vi "Get Page VI.vi"(8 "error in (no error)":errorcluster, 9 "GUID":string, 10 "Item Ref":T1 format="%.0x", 11 "System Explorer Dispatcher Implementation in":refnum<class "System Explorer Dispatcher.lvclass">) -> (0 "error out":errorcluster, 2 "page reference":refnum<vi>, 3 "System Explorer Dispatcher Implementation out":refnum<class "System Explorer Dispatcher.lvclass">)   [LabVIEW 2020, in "AIM ARINC 429 System Explorer.lvlib" / "Implementation.lvlib" / "System Explorer Dispatcher.lvclass"]
uses:
  System Explorer Dispatcher.lvclass
  <vilib>/NI VeriStand/Custom Device API/Custom Device Item Ref.ctl
  Scripting/AIM/Constants.vi
  System Explorer/Pages/Timing.vi
  Implementation.lvlib
  Scripting/AIM/AIM ARINC 429 Scripting.lvlib
  <vilib>/NI VeriStand/Custom Device API/Custom Device API.lvlib
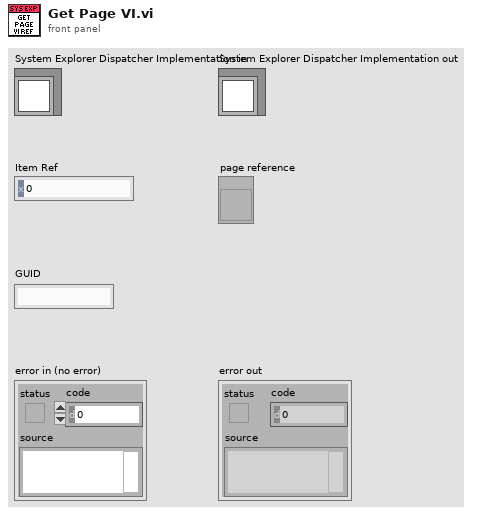
[diagram p1: front panel]
types:
  T1 = typedef "Custom Device API.lvlib/Custom Device Item Ref.ctl" = u64
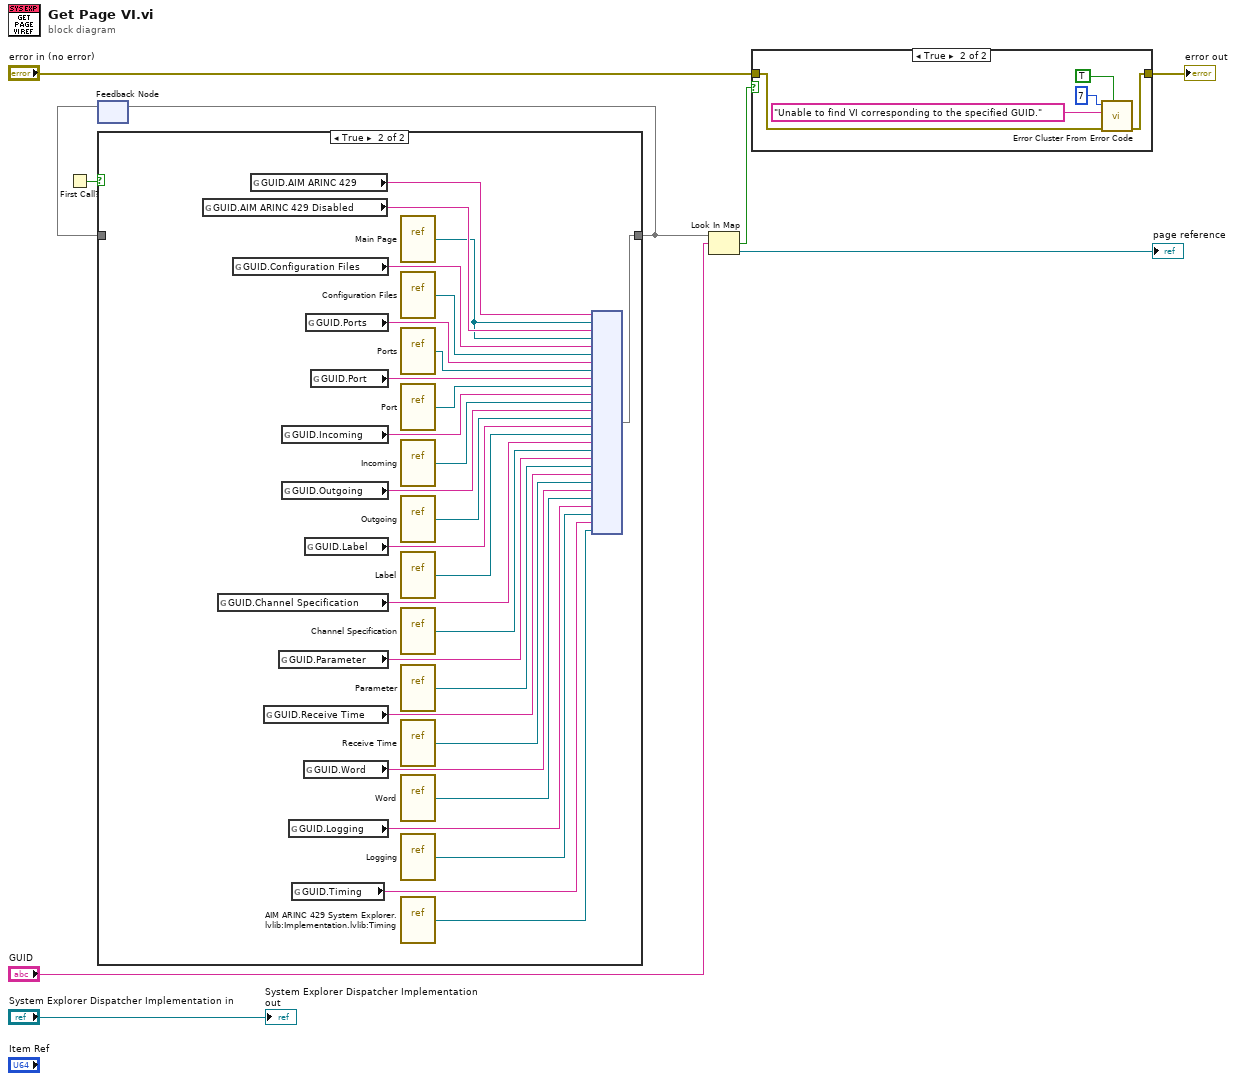
[diagram p0: block diagram]
diagram:
  n1 = First Call?() -> (First Call?: T/F=w8:bool)
  n2 = feedback #1() -> (w7:map{string, refnum<vi>})  [unwired: 1 in]
  n3 = case shown="True" w8 {
    tunnel: [w10 w38] -> w6
    tunnel: w7 -> [w10 _]
    frame False {
    }
    frame True {
      n4 = global read "Constants.vi" "GUID.AIM ARINC 429 Disabled"() -> (w16:string)
      n5 = global read "Constants.vi" "GUID.Channel Specification"() -> (w25:string)
      n6 = global read "Constants.vi" "GUID.Configuration Files"() -> (w36:string)
      n7 = global read "Constants.vi" "GUID.AIM ARINC 429"() -> (w17:string)
      n8 = global read "Constants.vi" "GUID.Receive Time"() -> (w21:string)
      n9 = global read "Constants.vi" "GUID.Parameter"() -> (w23:string)
      n10 = global read "Constants.vi" "GUID.Incoming"() -> (w31:string)
      n11 = global read "Constants.vi" "GUID.Outgoing"() -> (w29:string)
      n12 = global read "Constants.vi" "GUID.Logging"() -> (w14:string)
      n13 = global read "Constants.vi" "GUID.Timing"() -> (w12:string)
      n14 = global read "Constants.vi" "GUID.Word"() -> (w19:string)
      n15 = global read "Constants.vi" "GUID.Label"() -> (w27:string)
      n16 = global read "Constants.vi" "GUID.Ports"() -> (w35:string)
      n17 = global read "Constants.vi" "GUID.Port"() -> (w33:string)
      n18 = vi-ref "Main Page.vi"() -> (w15:refnum<vi>)
      n19 = vi-ref "Configuration Files.vi"() -> (w37:refnum<vi>)
      n20 = vi-ref "Ports.vi"() -> (w34:refnum<vi>)
      n21 = vi-ref "Port.vi"() -> (w32:refnum<vi>)
      n22 = vi-ref "Incoming.vi"() -> (w30:refnum<vi>)
      n23 = vi-ref "Outgoing.vi"() -> (w28:refnum<vi>)
      n24 = vi-ref "Label.vi"() -> (w26:refnum<vi>)
      n25 = vi-ref "Channel Specification.vi"() -> (w24:refnum<vi>)
      n26 = vi-ref "Parameter.vi"() -> (w22:refnum<vi>)
      n27 = vi-ref "Receive Time.vi"() -> (w20:refnum<vi>)
      n28 = vi-ref "Word.vi"() -> (w18:refnum<vi>)
      n29 = vi-ref "Logging.vi"() -> (w13:refnum<vi>)
      n30 = vi-ref "AIM ARINC 429 System Explorer.lvlib:Implementation.lvlib:Timing.vi"() -> (w11:refnum<vi>)
      n31 = node(w17, w15, w16, w15, w36, w37, w35, w34, w33, w32, w31, w30, w29, w28, w27, w26, w25, w24, w23, w22, w21, w20, w19, w18, w14, w13, w12, w11) -> (w38:map{string, refnum<vi>})
    }
  }
  n32 = feedback-in #1(w6) -> ()
  n33 = Look In Map(map=w6, key="GUID") -> (key not found?=w4:bool, value=→"page reference":refnum<vi>)  [unwired: 1 in]
  n34 = case shown="True" w4 {
    tunnel: [w39 w41] -> w3
    tunnel: "error in (no error)" -> [w39 w40]
    frame False {
    }
    frame True {
      n35 = call <vilib>:"Error Cluster From Error Code.vi"("show call chain? (False)"=TRUE, "error in (no error)"=w40, "error message (\"\")"="Unable to find VI corresponding to the specified GUID." ("error message (\"\")"), "error code (0)"=7) -> ("error out"=w41:errorcluster)  [unwired: 5 in]
    }
  }
  "error out" <- w3
  "System Explorer Dispatcher Implementation out" <- "System Explorer Dispatcher Implementation in"
